vi "Get Subscription Attributes.vi"(8 "error in (no error)":errorcluster, 11 "Subscription in":refnum<class "Subscription.lvclass">) -> (0 "error out":errorcluster, 2 "Subscription Attributes":T1[](array[typedef]), 3 "Subscription out":refnum<class "Subscription.lvclass">)   [LabVIEW 2015, in "NI_AWS_SNS.lvlib" / "Subscription.lvclass"]
doc: "Returns all of the properties of a subscription."
uses:
  Subscription.lvclass
  Subscription Attribute Value Pair.ctl
  Subscription Attribute.ctl
  Core/HTTP Request/Request Options.ctl
  Core/HTTP Request/Name Value Pair.ctl
  Core/HTTP Request/Region handling.ctl
  Core/HTTP Request/URL formatting.ctl
  Core/ARN/ARN.lvclass/ARN.ctl
  Core/ARN/Read ARN.vi
  Core/HTTP Request/HTTP Request.lvclass
  XML Parsing/NI_XML Parsing.lvlib
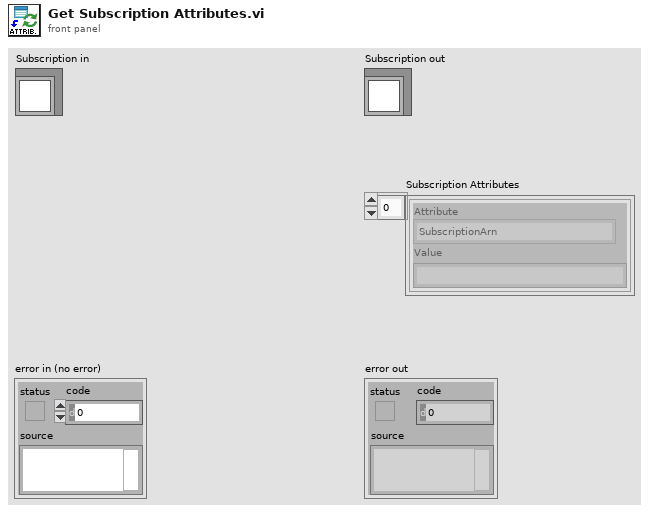
[diagram p1: front panel]
types:
  T1 = typedef "NI_AWS_SNS.lvlib/Subscription.lvclass/Subscription Attribute Value Pair.ctl" = cluster{"Attribute":T2, "Value":string}
  T2 = typedef "NI_AWS_SNS.lvlib/Subscription.lvclass/Subscription Attribute.ctl" = enum16{"SubscriptionArn", "TopicArn", "Owner", "ConfirmationWasAuthenticated", "DeliveryPolicy", "EffectiveDeliveryPolicy", "RawMessageDelivery", "Endpoint", "Protocol"}
  T3 = typedef "NI_AWS_Core.lvlib/HTTP Request.lvclass/Name Value Pair.ctl" = cluster{"name":string, "value":string}
  T4 = typedef "NI_AWS_Core.lvlib/HTTP Request.lvclass/Request Options.ctl" = cluster{"request headers":T3[], "request parameters":T3[], "request body":string, "region handling":T5, "URL formatting":T6}
  T5 = typedef "NI_AWS_Core.lvlib/HTTP Request.lvclass/Region handling.ctl" = enum16{"use region everywhere", "use region (authentication only)", "use region (URL only)", "ignore region everwhere"}
  T6 = typedef "NI_AWS_Core.lvlib/HTTP Request.lvclass/URL formatting.ctl" = enum16{"region-", "region."}
  T7 = typedef "NI_AWS_Core.lvlib/HTTP Request.lvclass/Response.ctl" = cluster{"Headers":string, "Body":string}
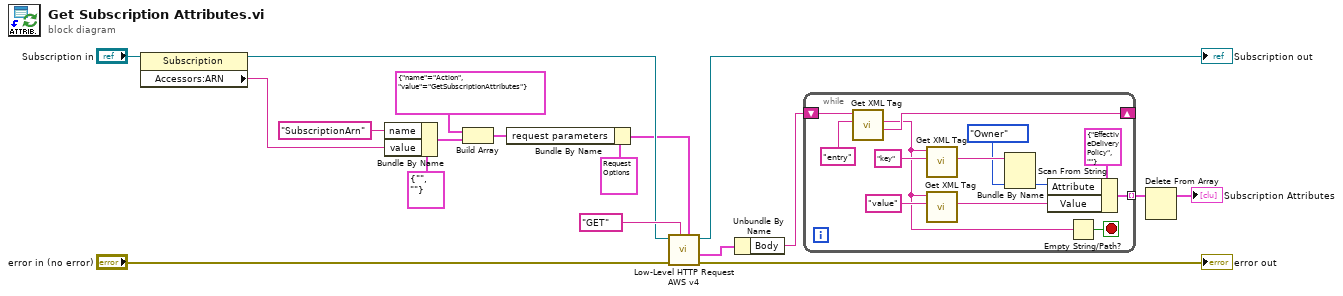
[diagram p0: block diagram]
diagram:
  n1 = property class="Subscription"(reference="Subscription in") -> (reference out=w3:refnum<class "Subscription.lvclass">, "Accessors:ARN"=w6:string)  [unwired: 1 in, 1 out]
  n2 = Bundle By Name(cluster=T3 {"name"="", "value"=""} ("Name Value Pair"), "name"="SubscriptionArn", "value"=w6) -> (w8:T3)
  n3 = Build Array(T3 {"name"="Action", "value"="GetSubscriptionAttributes"} ("Name Value Pair"), w8) -> (w11:T3[])
  n4 = Bundle By Name(cluster=T4 {"request headers"=[], "request parameters"=[], "request body"="", "region handling"=enum."use region everywhere", "URL formatting"=enum."region."} ("Request Options"), "request parameters"=w11) -> (w1:T4)
  n5 = call "Low-Level HTTP Request AWS v4.vi"("Request Options"=w1, "HTTP-Verb"="GET", "error in (no error)"="error in (no error)", "AWS Core in"=w3) -> ("error out"=→"error out":errorcluster, "Response"=w5:T7, "AWS Core out"=→"Subscription out":refnum<class "Subscription.lvclass">)  [unwired: 4 in, 1 out]
  n6 = Unbundle By Name(w5) -> ("Body"=w17:string)
  n7 = while {
    shift-right: [w30] -> _
    shift-left: w17 -> [w31]
    tunnel: [w25] -> w16 mode=indexing
    stop <- w23 stop-if-true
    n8 = call "Get XML Tag.vi"("Tag name"="entry", "XML String in"=w31) -> ("Remaining string"=w30:string, "Tag value"=w24:string)  [unwired: 5 in, 3 out]
    n9 = call "Get XML Tag.vi"("Tag name"="key", "XML String in"=w24) -> ("Tag value"=w22:string)  [unwired: 5 in, 4 out]
    n10 = call "Get XML Tag.vi"("Tag name"="value", "XML String in"=w24) -> ("Tag value"=w26:string)  [unwired: 5 in, 4 out]
    n11 = Scan From String(input string=w22, default 1=Subscription_Attribute."Owner" ("Attribute")) -> (output 1=w21:T2)  [unwired: 3 in, 3 out]
    n12 = Bundle By Name(cluster=T1 {"Attribute"=enum."EffectiveDeliveryPolicy", "Value"=""} ("Subscription Attribute Value Pair"), "Attribute"=w21, "Value"=w26) -> (w25:T1)
    n13 = Empty String/Path?(string/path=w24) -> (empty?=w23:bool)
  }
  n14 = Delete From Array(array=w16) -> (array with subset deleted=→"Subscription Attributes":T1[])  [unwired: 2 in, 1 out]
